vi "Set_Operation_Mode.vi"(8 "error in (no error)":errorcluster, 10 "Motor Control Mode":T1, 11 "ServoDrive in":refnum<class "ServoDrive.lvclass">) -> (0 "error out":errorcluster, 3 "ServoDrive out":refnum<class "ServoDrive.lvclass">)   [LabVIEW 2021, in "ServoDrive.lvclass"]
uses:
  ServoDrive.lvclass
  Motor/Type_Defs/Control_Mode.ctl
  ServoDrive.lvclass/ServoDrive.ctl
  Motor/Motor.lvclass
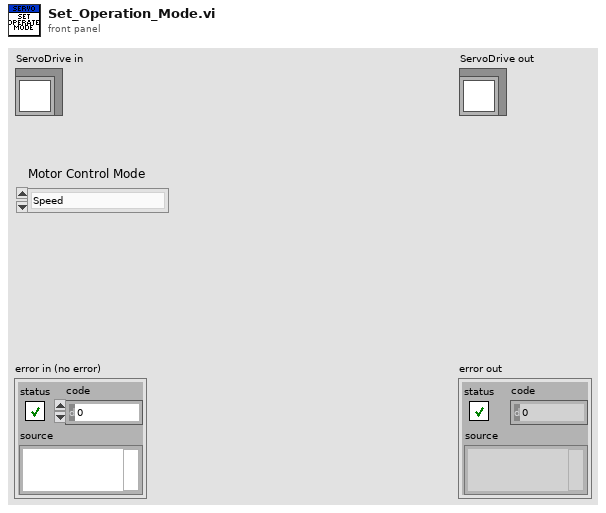
[diagram p1: front panel]
types:
  T1 = typedef "Motor.lvclass/Control_Mode.ctl" = enum16{"Speed", "Torque"}
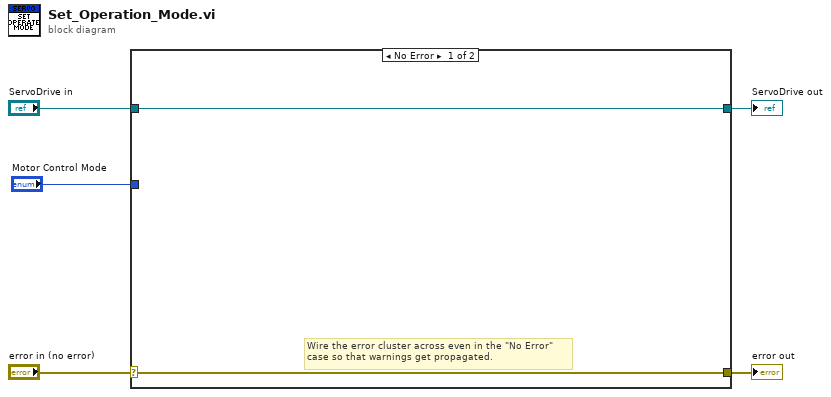
[diagram p0: block diagram]
diagram:
  n1 = case shown="No Error" "error in (no error)" {
    selector: "error in (no error)" -> [w6 w9]
    tunnel: [w6 w9] -> w4
    tunnel: [w7 w8] -> w2
    tunnel: "ServoDrive in" -> [w7 w8]
    tunnel: "Motor Control Mode" -> [_ _]
    frame No Error {
      # "Wire the error cluster across even in the \"No Error\"\ncase so that warnings get propagated."
    }
    frame Error {
    }
  }
  "error out" <- w4
  "ServoDrive out" <- w2
